vi "onTestExecution.vi"(6 "timeout (2000 ms)":i32=2000, 7 "Name":string, 8 "error in (no error)":errorcluster, 11 "Test Runner in":refnum<class "Test Runner.lvclass">) -> (0 "error out":errorcluster, 3 "Test Runner out":refnum<class "Test Runner.lvclass">)   [LabVIEW 2020, in "Caraya.lvlib" / "Test Runner.lvclass"]
uses:
  Test Runner.lvclass
  Assert/Assert Not Error.vi
  Test/Test.lvclass
  Assert/Assert.lvclass
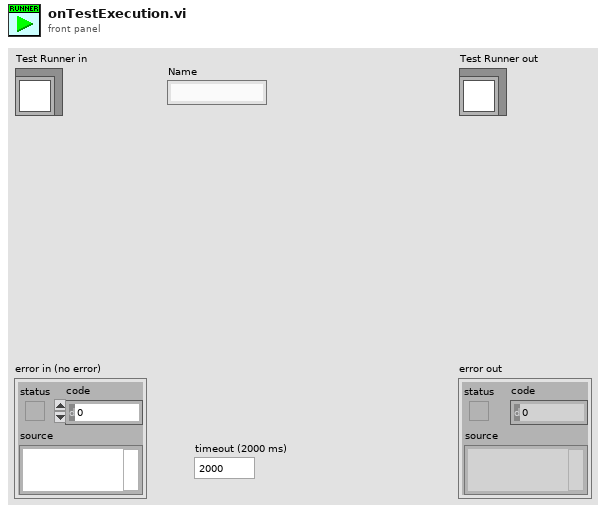
[diagram p1: front panel]
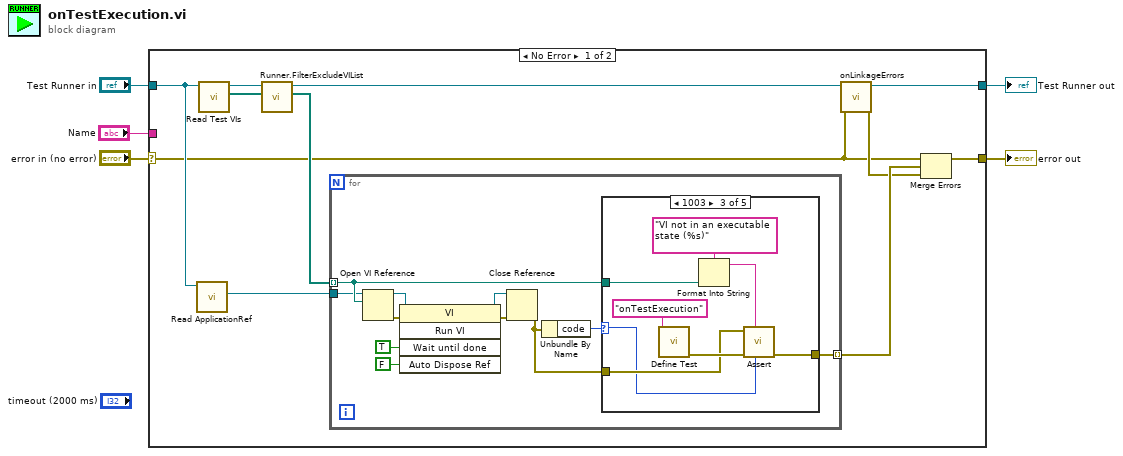
[diagram p0: block diagram]
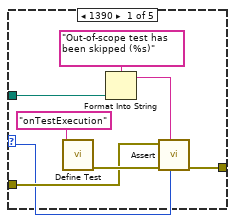
[diagram p2: hidden frame]
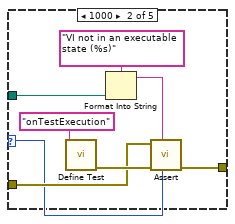
[diagram p3: hidden frame]
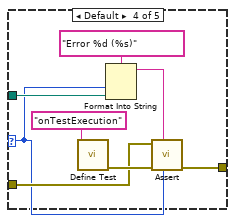
[diagram p4: hidden frame]
diagram:
  n1 = case shown="No Error" "error in (no error)" {
    selector: "error in (no error)" -> [w6 w62]
    tunnel: "Test Runner in" -> [w8 w61]
    tunnel: [w14 w61] -> w4
    tunnel: [w13 w62] -> w3
    tunnel: "Name" -> [_ _]
    frame No Error {
      n2 = call "Read ApplicationRef.vi"("Test Runner in"=w8) -> ("Application"=w15:refnum<vi>)  [unwired: 8 in, 2 out]
      n3 = call "Read Test VIs.vi"("Test Runner in"=w8) -> ("Test VIs"=w10:path[], "Test Runner out"=w7:refnum<class "Test Runner.lvclass">)  [unwired: 8 in, 1 out]
      n4 = call "Runner.FilterExcludeVIList.vi"("Paths"=w10, "Test Runner"=w7) -> ("Filtered Paths"=w9:path[], "Test Runner"=w11:refnum<class "Test Runner.lvclass">)  [unwired: 8 in]
      n5 = for {
        tunnel: w9 -> [w27] mode=indexing
        tunnel: [w26] -> w16 mode=indexing
        tunnel: w15 -> [w25]
        n6 = Open VI Reference(application reference (local)=w25, vi path=w27) -> (vi reference=w17:refnum<vi>, error out=w24:errorcluster)  [unwired: 4 in]
        n7 = invoke on="Invoke Node" class="VI" method="Run VI"(reference=w17, error in=w24, "Wait until done"=TRUE ("Wait Until Done"), "Auto Dispose Ref"=FALSE ("Auto Dispose Reference")) -> (reference out=w20:refnum<vi>, error out=w19:errorcluster)  [unwired: 1 in, 3 out]
        n8 = Close Reference(reference=w20, error in (no error)=w19) -> (error out=w18:errorcluster)
        n9 = Unbundle By Name(w18) -> ("code"=w21:i32)
        n10 = case shown="1003" w21 {
          selector: w21 -> [w28 w36 w44 w52 _]
          tunnel: w18 -> [w29 w37 w45 w53 w60]
          tunnel: [w31 w39 w47 w56 w60] -> w26
          tunnel: w27 -> [w35 w43 w51 w59 _]
          frame 1390 {
            n11 = call "Define Test.vi"("Label (VI Title)"="onTestExecution" ("Label")) -> ("error out"=w32:errorcluster)  [unwired: 9 in, 1 out]
            n12 = Format Into String(format string="Out-of-scope test has been skipped (%s)" ("Label"), w35) -> (resulting string=w30:string)  [unwired: 2 in, 1 out]
            n13 = call-poly "Assert.vi"("error code (1)"=w28, "Label"=w30, "error in (no error)"=w32, "Not Error?"=w29) -> ("error out"=w31:errorcluster)  [unwired: 6 in, 1 out]
          }
          frame 1000 {
            n14 = call "Define Test.vi"("Label (VI Title)"="onTestExecution" ("Label")) -> ("error out"=w40:errorcluster)  [unwired: 9 in, 1 out]
            n15 = Format Into String(format string="VI not in an executable state (%s)" ("Label"), w43) -> (resulting string=w38:string)  [unwired: 2 in, 1 out]
            n16 = call-poly "Assert.vi"("error code (1)"=w36, "Label"=w38, "error in (no error)"=w40, "Not Error?"=w37) -> ("error out"=w39:errorcluster)  [unwired: 6 in, 1 out]
          }
          frame 1003 {
            n17 = call "Define Test.vi"("Label (VI Title)"="onTestExecution" ("Label")) -> ("error out"=w48:errorcluster)  [unwired: 9 in, 1 out]
            n18 = Format Into String(format string="VI not in an executable state (%s)" ("Label"), w51) -> (resulting string=w46:string)  [unwired: 2 in, 1 out]
            n19 = call-poly "Assert.vi"("error code (1)"=w44, "Label"=w46, "error in (no error)"=w48, "Not Error?"=w45) -> ("error out"=w47:errorcluster)  [unwired: 6 in, 1 out]
          }
          frame Default {
            n20 = call "Define Test.vi"("Label (VI Title)"="onTestExecution" ("Label")) -> ("error out"=w54:errorcluster)  [unwired: 9 in, 1 out]
            n21 = Format Into String(format string="Error %d (%s)" ("Label"), w52, w59) -> (resulting string=w55:string)  [unwired: 2 in, 1 out]
            n22 = call-poly "Assert.vi"("error code (1)"=w52, "Label"=w55, "error in (no error)"=w54, "Not Error?"=w53) -> ("error out"=w56:errorcluster)  [unwired: 6 in, 1 out]
          }
          frame 0 {
          }
        }
      }
      n23 = call-dynamic "onLinkageErrors.vi"("error in (no error)"=w6, "Test Runner in"=w11) -> ("error out"=w12:errorcluster, "Test Runner out"=w14:refnum<class "Test Runner.lvclass">)  [unwired: 8 in]
      n24 = Merge Errors(w6, w16, w12) -> (w13:errorcluster)
    }
    frame Error {
    }
  }
  "error out" <- w3
  "Test Runner out" <- w4
